vi "Titles.vi"() -> (0 "数据及Titles":cluster{"Titles":string[], "温度相关数据":T1})   [LabVIEW 2026, in "Data Collection and Save.lvlib"]
uses:
  Data Collection and Save.lvlib
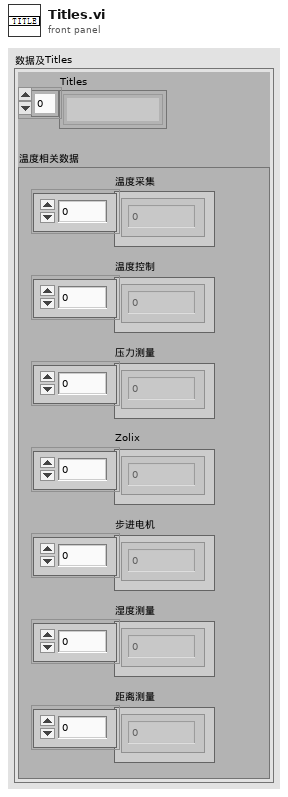
[diagram p1: front panel]
types:
  T1 = typedef "全局变量数据.ctl" = cluster{"温度采集":dbl[], "温度控制":dbl[], "压力测量":dbl[], "Zolix":dbl[], "步进电机":dbl[], "湿度测量":dbl[], "距离测量":dbl[]}
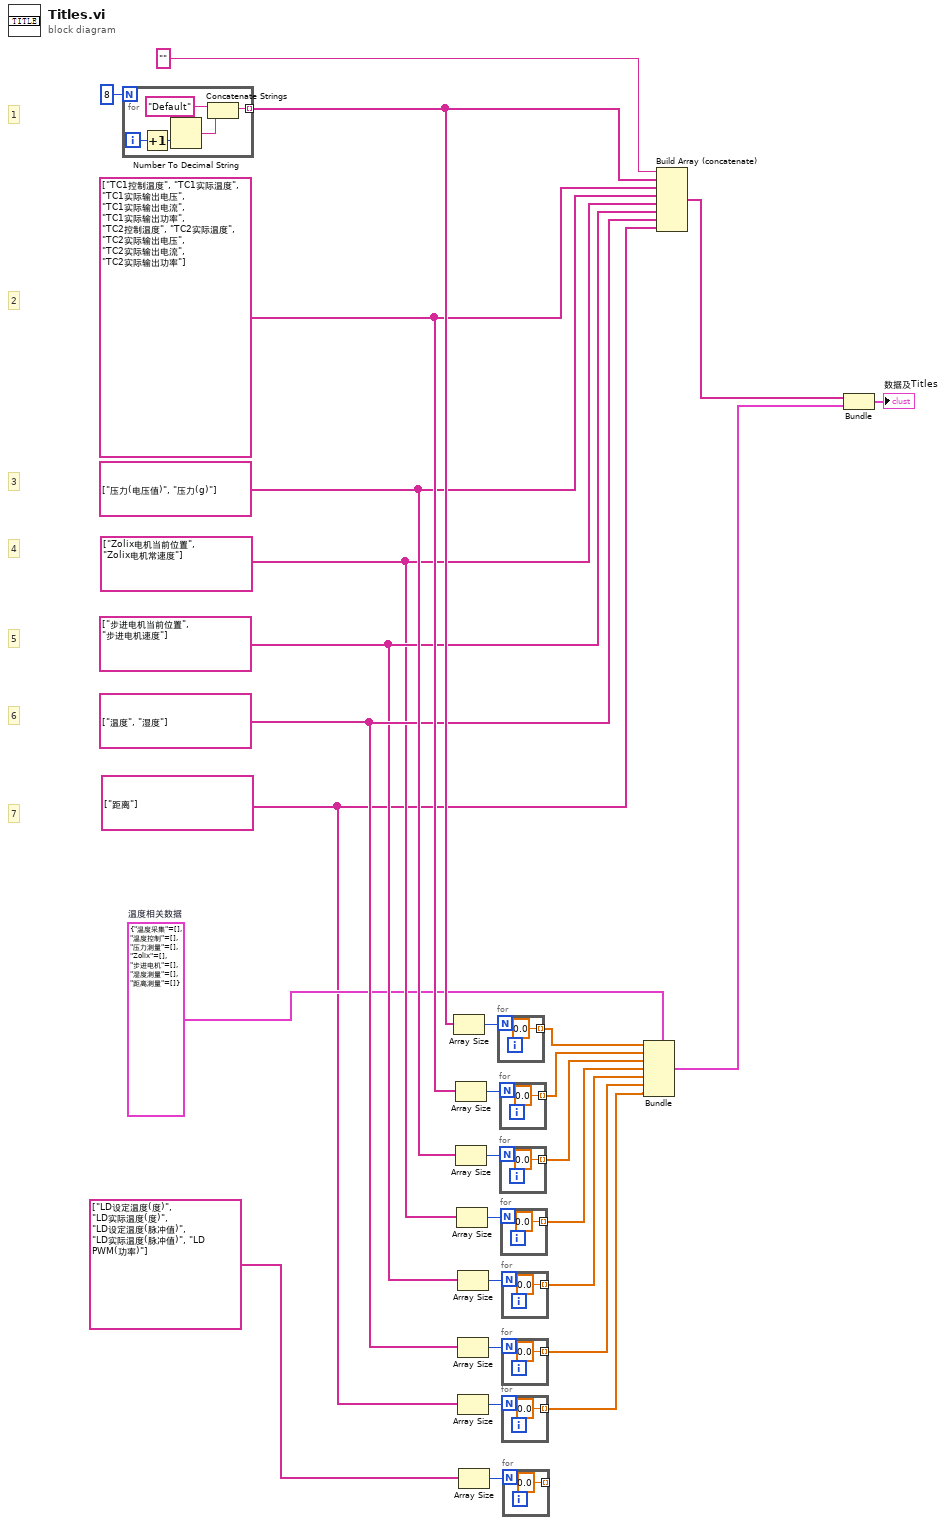
[diagram p0: block diagram]
diagram:
  w2 = string[] ["距离"]
  w5 = T1 {"温度采集"=[], "温度控制"=[], "压力测量"=[], "Zolix"=[], "步进电机"=[], "湿度测量"=[], "距离测量"=[]}  # 温度相关数据
  w7 = string[] ["步进电机当前位置", "步进电机速度"]
  w6 = string[] ["Zolix电机当前位置", "Zolix电机常速度"]
  w14 = string[] ["温度", "湿度"]
  w21 = string[] ["压力(电压值)", "压力(g)"]
  w23 = string[] ["TC1控制温度", "TC1实际温度", "TC1实际输出电压", "TC1实际输出电流", "TC1实际输出功率", "TC2控制温度", "TC2实际温度", "TC2实际输出电压", "TC2实际输出电流", "TC2实际输出功率"]
  # "7"
  # "6"
  # "5"
  # "4"
  # "3"
  # "2"
  # "1"
  n1 = for {
    N: 8 -> [_]
    tunnel: [w30] -> w25 mode=indexing
    i -> [w34]
    n2 = Increment(x=w34) -> (x+1=w33:i32)
    n3 = Number To Decimal String(number=w33) -> (decimal integer string=w32:string)  [unwired: 1 in]
    n4 = Concatenate Strings("Default", w32) -> (w30:string)
  }
  n5 = Array Size(array=w25) -> (size(s)=w27:i32)
  n6 = Array Size(array=w23) -> (size(s)=w24:i32)
  n7 = Array Size(array=w21) -> (size(s)=w22:i32)
  n8 = Array Size(array=w6) -> (size(s)=w18:i32)
  n9 = Array Size(array=w7) -> (size(s)=w9:i32)
  n10 = Array Size(array=w14) -> (size(s)=w16:i32)
  n11 = Array Size(array=w2) -> (size(s)=w4:i32)
  n12 = Array Size(array=string[] ["LD设定温度(度)", "LD实际温度(度)", "LD设定温度(脉冲值)", "LD实际温度(脉冲值)", "LD PWM(功率)"]) -> (size(s)=w13:i32)
  n13 = for {
    N: w27 -> [_]
    tunnel: [0.0] -> w26 mode=indexing
  }
  n14 = for {
    N: w24 -> [_]
    tunnel: [0.0] -> w20 mode=indexing
  }
  n15 = for {
    N: w22 -> [_]
    tunnel: [0.0] -> w19 mode=indexing
  }
  n16 = for {
    N: w18 -> [_]
    tunnel: [0.0] -> w17 mode=indexing
  }
  n17 = for {
    N: w9 -> [_]
    tunnel: [0.0] -> w8 mode=indexing
  }
  n18 = for {
    N: w16 -> [_]
    tunnel: [0.0] -> w15 mode=indexing
  }
  n19 = for {
    N: w4 -> [_]
    tunnel: [0.0] -> w3 mode=indexing
  }
  n20 = for {
    N: w13 -> [_]
    tunnel: [0.0] -> _ mode=indexing
  }
  n21 = Bundle(cluster=w5, "温度采集"=w26, "温度控制"=w20, "压力测量"=w19, "Zolix"=w17, "步进电机"=w8, "湿度测量"=w15, "距离测量"=w3) -> (w10:T1)
  n22 = Build Array (concatenate)("" ("元素"), w25, w23, w21, w6, w7, w14, w2) -> (w11:string[])
  n23 = Bundle(w11, "温度相关数据"=w10) -> (→"数据及Titles":cluster{string[], "温度相关数据":T1})  [unwired: 1 in]
